vi "Set Context.vi"(8 "error in (no error)":errorcluster, 10 "Process Context":refnum<class "Process.lvclass">, 11 "Process In":refnum<class "Process.lvclass">) -> (0 "error out":errorcluster, 3 "Process Out":refnum<class "Process.lvclass">)   [LabVIEW 2020, in "Process.lvclass"]
doc: "Framework method for setting the context of a process. Any process added to an application automatically gets the correct context by the framework and using this method is not necessary."
uses:
  Process.lvclass
  Process.lvclass/Process.ctl
  <vilib>/Utility/error.llb/Clear Errors.vi
  <vilib>/Utility/error.llb/Error Cluster From Error Code.vi
  <vilib>/ErrorRing/Error Ring.xnode
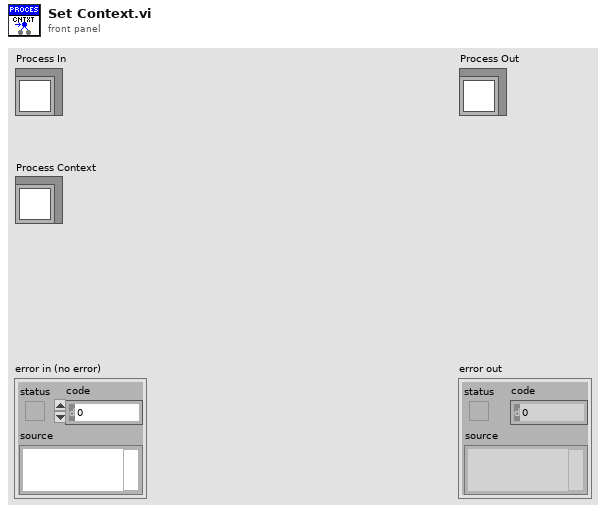
[diagram p1: front panel]
types:
  T1 = typedef "Process.lvclass/Lifecycle State.ctl" = enum16{"Uninitialized", "Initialized", "Started", "Running", "Stopped", "Finished"}
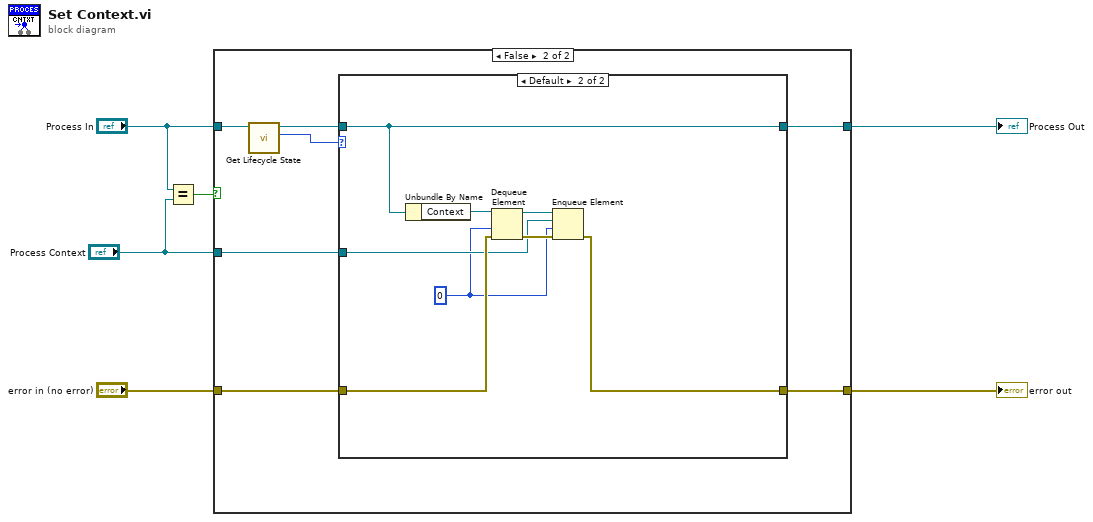
[diagram p0: block diagram]
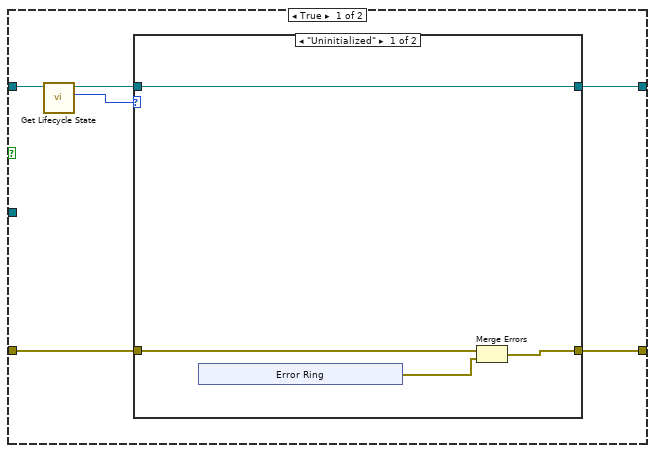
[diagram p2: hidden frame]
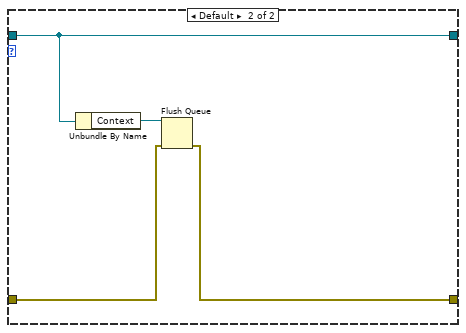
[diagram p3: hidden frame]
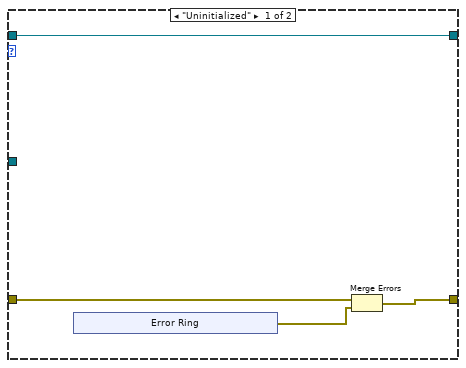
[diagram p4: hidden frame]
diagram:
  n1 = Equal?(x="Process In", y="Process Context") -> (x = y?=w1:bool)
  n2 = case shown="False" w1 {
    tunnel: [w12 w31] -> w6
    tunnel: [w11 w30] -> w5
    tunnel: "error in (no error)" -> [w8 w27]
    tunnel: "Process In" -> [w7 w26]
    tunnel: "Process Context" -> [_ w25]
    frame True {
      n3 = call "Get Lifecycle State.vi"("Process In"=w7) -> ("Lifecycle State"=w9:T1, "Process Out"=w10:refnum<class "Process.lvclass">)  [unwired: 7 in, 2 out]
      n4 = case shown="\"Uninitialized\"" w9 {
        tunnel: [w16 w24] -> w12
        tunnel: [w14 w22] -> w11
        tunnel: w10 -> [w16 w24]
        tunnel: w8 -> [w15 w21]
        frame "Uninitialized" {
          n5 = xnode "Error Ring"() -> ("error out"=w13:errorcluster)
          n6 = Merge Errors(w15, w13) -> (w14:errorcluster)
        }
        frame Default {
          n7 = Unbundle By Name(w24) -> ("Context"=w23:refnum<queue>)
          n8 = Flush Queue(queue=w23, error in (no error)=w21) -> (error out=w22:errorcluster)  [unwired: 2 out]
        }
      }
    }
    frame False {
      n9 = call "Get Lifecycle State.vi"("Process In"=w26) -> ("Lifecycle State"=w28:T1, "Process Out"=w29:refnum<class "Process.lvclass">)  [unwired: 7 in, 2 out]
      n10 = case shown="Default" w28 {
        tunnel: [w35 w47] -> w31
        tunnel: [w33 w43] -> w30
        tunnel: w25 -> [_ w41]
        tunnel: w29 -> [w35 w47]
        tunnel: w27 -> [w34 w42]
        frame "Uninitialized" {
          n11 = xnode "Error Ring"() -> ("error out"=w32:errorcluster)
          n12 = Merge Errors(w34, w32) -> (w33:errorcluster)
        }
        frame Default {
          w40 = 0 ("timeout in ms (-1)")
          n13 = Unbundle By Name(w47) -> ("Context"=w46:refnum<queue>)
          n14 = Dequeue Element(queue=w46, timeout in ms (-1)=w40, error in (no error)=w42) -> (queue out=w45:refnum<queue>, error out=w44:errorcluster)  [unwired: 2 out]
          n15 = Enqueue Element(queue=w45, element=w41, timeout in ms (-1)=w40, error in (no error)=w44) -> (error out=w43:errorcluster)  [unwired: 2 out]
        }
      }
    }
  }
  "error out" <- w5
  "Process Out" <- w6
